vi "constant-concatenate-command.vi"(11 "error in":errorcluster) -> (15 "error out":errorcluster)   [LabVIEW 2024]
doc: "Static SAST fixture: two constants are concatenated into System Exec command line. Do not run."
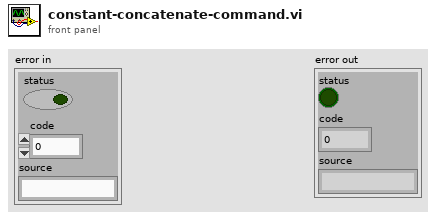
[diagram p1: front panel]
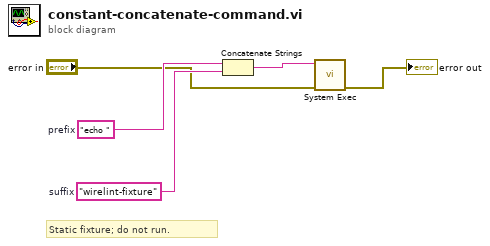
[diagram p0: block diagram]
diagram:
  w3 = "wirelint-fixture"  # suffix
  w2 = "echo "  # prefix
  # "Static fixture; do not run."
  n1 = Concatenate Strings(w2, w3) -> (w4:string)
  n2 = call <vilib>:"System Exec.vi"("error in (no error)"="error in", "command line"=w4) -> ("error out"=→"error out":errorcluster)  [unwired: 6 in, 3 out]
